vi "FGV-BroadcastRegistry.vi"(0 "Source":string, 5 "Target":string, 7 "Status":string, 9 "API":string, 11 "Error In":errorcluster caption="error in (no error)", 12 "Operation":T3) -> (4 "Response Message":string[](array[string]), 6 "Values":T1[](array[typedef]), 15 "error out":errorcluster)   [LabVIEW 2017, in "Communicable State Machine.lvlib"]
doc: "### FGV-BroadcastRegistry.vi\n\n-- <b>Controls</b> --\n- <b>Source</b>:\n- <b>Target</b>:\n- <b>Status</b>:\n- <b>API</b>:\n- <b>Operation</b>:\n\n-- <b>Indicators</b> --\n- <b>response message</b>:"
uses:
  Communicable State Machine.lvlib
  Operation-BroadcastRegistry.ctl
  BroadcastRegistry/BroadcastRegistry-Value.ctl
  AdvanceAPI/CSM - Broadcast Message Type.ctl
  BroadcastRegistry/BroadcastRegistry.ctl
  ChangeFlag/ChangeFlag-Write.vi
  Utility/Random Change Flag.vi
  ChangeFlag/ChangeFlagDB.vi
  _Shared/CSM Shared.lvlib
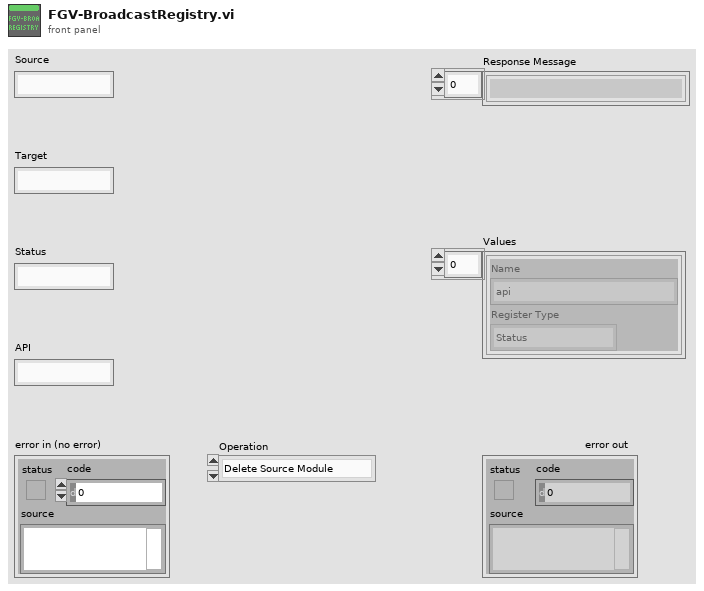
[diagram p1: front panel]
types:
  T1 = typedef "Communicable State Machine.lvlib/BroadcastRegistry-Value.ctl" = cluster{"Name":string, "Register Type":T2}
  T2 = typedef "Communicable State Machine.lvlib/CSM - Broadcast Message Type.ctl" = enum16{"<Null>", "Status", "Interrupt"}
  T3 = typedef "Communicable State Machine.lvlib/Operation-BroadcastRegistry.ctl" = enum16{"Delete Source Module", "Delete Target Module", "Remove Module", "Register", "Unregister", "Check", "List Status", "List Entries", "List Status Of Source", "Drop", "Register As Status", "Register As Interrupt"}
  T4 = typedef "Communicable State Machine.lvlib/BroadcastRegistry.ctl" = cluster{"RegistryTable":variant}
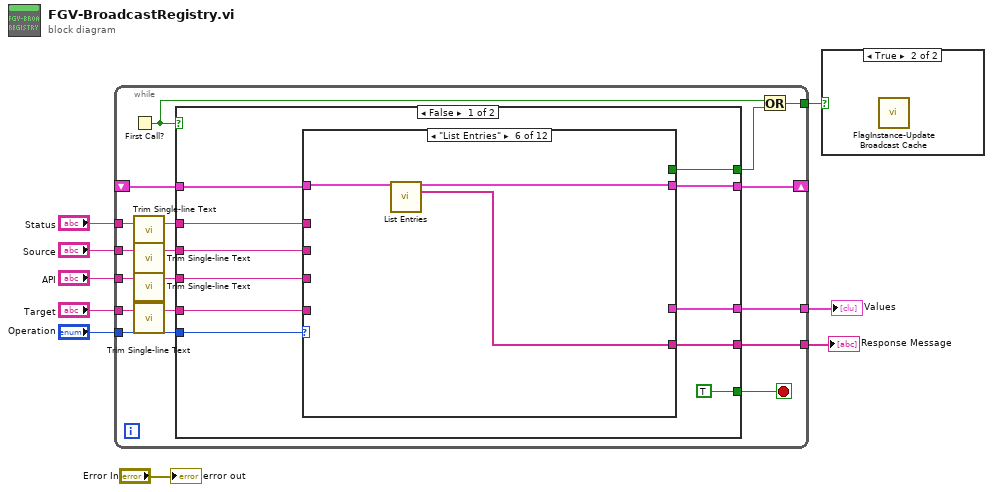
[diagram p0: block diagram]
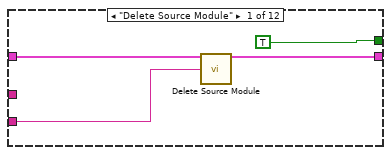
[diagram p2: hidden frame]
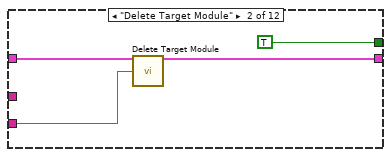
[diagram p3: hidden frame]
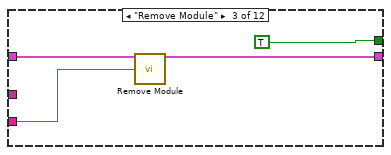
[diagram p4: hidden frame]
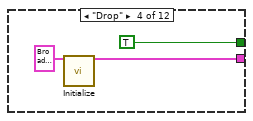
[diagram p5: hidden frame]
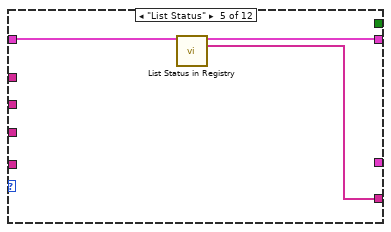
[diagram p6: hidden frame]
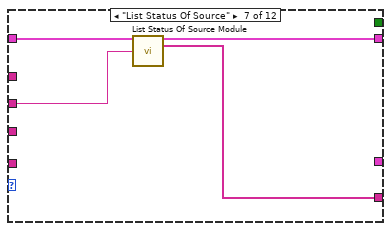
[diagram p7: hidden frame]
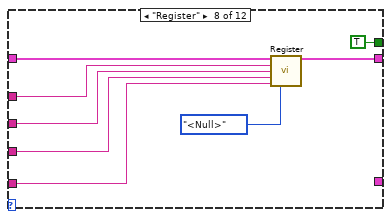
[diagram p8: hidden frame]
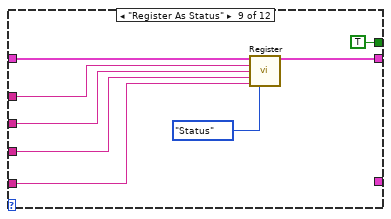
[diagram p9: hidden frame]
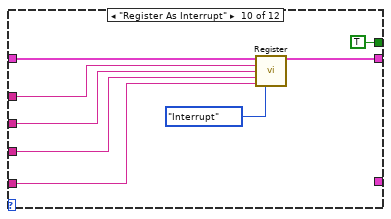
[diagram p10: hidden frame]
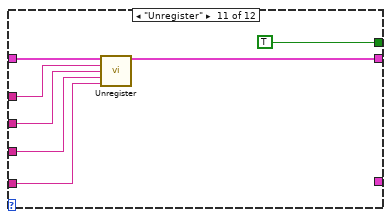
[diagram p11: hidden frame]
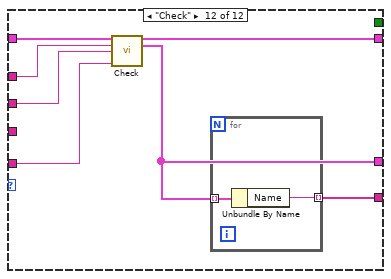
[diagram p12: hidden frame]
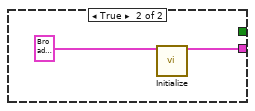
[diagram p13: hidden frame]
diagram:
  n1 = while {
    shift-right: [w25] -> _
    shift-left: _ -> [w24]
    tunnel: "Operation" -> [w23]
    tunnel: "Target" -> [w16]
    tunnel: "Source" -> [w15]
    tunnel: "Status" -> [w17]
    tunnel: "API" -> [w18]
    tunnel: [w22] -> w1
    tunnel: [w19] -> w3
    tunnel: [w10] -> w2
    stop <- w26 stop-if-true
    n2 = First Call?() -> (First Call?: T/F=w20:bool)
    n3 = call "Trim Single-line Text.vi"("single-line text"=w17) -> ("trimed text"=w12:string)  [unwired: 2 in]
    n4 = call "Trim Single-line Text.vi"("single-line text"=w15) -> ("trimed text"=w14:string)  [unwired: 2 in]
    n5 = call "Trim Single-line Text.vi"("single-line text"=w18) -> ("trimed text"=w11:string)  [unwired: 2 in]
    n6 = call "Trim Single-line Text.vi"("single-line text"=w16) -> ("trimed text"=w13:string)  [unwired: 2 in]
    n7 = case shown="False" w20 {
      tunnel: [TRUE _] -> w26
      tunnel: [w28 w104] -> w25
      tunnel: w24 -> [w29 _]
      tunnel: w23 -> [w36 _]
      tunnel: w13 -> [w35 _]
      tunnel: w14 -> [w34 _]
      tunnel: w12 -> [w33 _]
      tunnel: w11 -> [w32 _]
      tunnel: [w31 _] -> w22
      tunnel: [w30 _] -> w21
      tunnel: [w27 _] -> w10
      frame False {
        n8 = case shown="\"List Entries\"" w36 {
          tunnel: [w39 w43 w47 w50 w54 w57 w61 w69 w77 w85 w91 w99] -> w28
          tunnel: w29 -> [w40 w44 w48 _ w55 w58 w62 w68 w76 w84 w92 w100]
          tunnel: w35 -> [_ _ _ _ _ _ _ w64 w72 w80 w88 w98]
          tunnel: w34 -> [w38 w42 w46 _ _ _ w60 w66 w74 w82 w89 w97]
          tunnel: w33 -> [_ _ _ _ _ _ _ w67 w75 w83 w90 w96]
          tunnel: w32 -> [_ _ _ _ _ _ _ w65 w73 w81 w87 _]
          tunnel: [_ _ _ _ w53 w56 w59 _ _ _ _ w94] -> w31
          tunnel: [TRUE ("Cache changed?") TRUE ("Cache changed?") TRUE ("Cache changed?") TRUE ("Cache changed?") _ _ _ TRUE ("Cache changed?") TRUE ("Cache changed?") TRUE ("Cache changed?") TRUE ("Cache changed?") _] -> w30
          tunnel: [_ _ _ _ _ _ _ _ _ _ _ w95] -> w27
          frame "Delete Source Module" {
            n9 = call "Delete Source Module.vi"("BroadcastRegistry In"=w40, "SourceCSM"=w38) -> ("BroadcastRegistry Out"=w39:T4)  [unwired: 13 in]
          }
          frame "Delete Target Module" {
            n10 = call "Delete Target Module.vi"("BroadcastRegistry In"=w44, "TargetCSM"=w42) -> ("BroadcastRegistry Out"=w43:T4)  [unwired: 13 in]
          }
          frame "Remove Module" {
            n11 = call "Remove Module.vi"("BroadcastRegistry In"=w48, "Source"=w46) -> ("BroadcastRegistry Out"=w47:T4)  [unwired: 13 in]
          }
          frame "Drop" {
            n12 = call "Initialize.vi"("BroadcastRegistry In"=T4 {"RegistryTable"=variant}) -> ("BroadcastRegistry Out"=w50:T4)  [unwired: 14 in]
          }
          frame "List Status" {
            n13 = call "List Status in Registry.vi"("BroadcastRegistry In"=w55) -> ("BroadcastRegistry Out"=w54:T4, "Broadcast"=w53:string[])  [unwired: 13 in]
          }
          frame "List Entries" {
            n14 = call "List Entries.vi"("BroadcastRegistry In"=w58) -> ("BroadcastRegistry Out"=w57:T4, "Array"=w56:string[])  [unwired: 13 in]
          }
          frame "List Status Of Source" {
            n15 = call "List Status Of Source Module.vi"("BroadcastRegistry In"=w62, "SourceCSM"=w60) -> ("BroadcastRegistry Out"=w61:T4, "Broadcast"=w59:string[])  [unwired: 12 in]
          }
          frame "Register" {
            n16 = call "Register.vi"("BroadcastRegistry In"=w68, "Broadcast"=w67, "SourceCSM"=w66, "Name"=w65, "TargetCSM"=w64, "Register Type"=CSM_-_Broadcast_Message_Type."<Null>") -> ("BroadcastRegistry Out"=w69:T4)  [unwired: 9 in]
          }
          frame "Register As Status" {
            n17 = call "Register.vi"("BroadcastRegistry In"=w76, "Broadcast"=w75, "SourceCSM"=w74, "Name"=w73, "TargetCSM"=w72, "Register Type"=CSM_-_Broadcast_Message_Type."Status") -> ("BroadcastRegistry Out"=w77:T4)  [unwired: 9 in]
          }
          frame "Register As Interrupt" {
            n18 = call "Register.vi"("BroadcastRegistry In"=w84, "Broadcast"=w83, "SourceCSM"=w82, "Name"=w81, "TargetCSM"=w80, "Register Type"=CSM_-_Broadcast_Message_Type."Interrupt") -> ("BroadcastRegistry Out"=w85:T4)  [unwired: 9 in]
          }
          frame "Unregister" {
            n19 = call "Unregister.vi"("BroadcastRegistry In"=w92, "Broadcast"=w90, "SourceCSM"=w89, "API"=w87, "TargetCSM"=w88) -> ("BroadcastRegistry Out"=w91:T4)  [unwired: 10 in]
          }
          frame "Check" {
            n20 = call "Check.vi"("BroadcastRegistry In"=w100, "Broadcast"=w96, "SourceCSM"=w97, "TargetCSM"=w98) -> ("BroadcastRegistry Out"=w99:T4, "Response Message Info"=w95:T1[])  [unwired: 10 in]
            n21 = for {
              tunnel: w95 -> [w102] mode=indexing
              tunnel: [w101] -> w94 mode=indexing
              n22 = Unbundle By Name(w102) -> ("Name"=w101:string)
            }
          }
        }
      }
      frame True {
        n23 = call "Initialize.vi"("BroadcastRegistry In"=T4 {"RegistryTable"=variant}) -> ("BroadcastRegistry Out"=w104:T4)  [unwired: 14 in]
      }
    }
    n24 = Or(x=w20, y=w21) -> (x .or. y?=w19:bool)
  }
  "Response Message" <- w1
  "Values" <- w2
  n25 = case shown="True" w3 {
    frame False {
    }
    frame True {
      n26 = call "FlagInstance-Update Broadcast Cache.vi"() -> ()  [unwired: 10 in, 2 out]
    }
  }
  "error out" <- "Error In"
